vi "Resolve Type.vi"(8 "error in":errorcluster, 11 "Type Name":string) -> (0 "error out":errorcluster, 3 "Runtime Type":refnum<k24>)   [LabVIEW 2026, in "ToastNotification.lvlib" / "Reflection DotNet.lvlib"]
doc: "Resolve a runtime type by its assembly-qualified name using System.Type.GetType(name, true). Skipped on incoming error. The caller owns the returned System.Type reference. WinRT names can include ContentType=WindowsRuntime."
uses:
  Reflection DotNet.lvlib
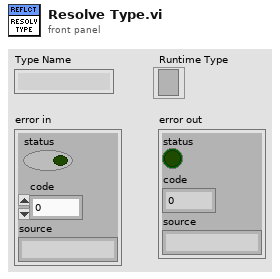
[diagram p1: front panel]
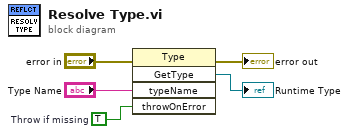
[diagram p0: block diagram]
diagram:
  w1 = TRUE  # Throw if missing
  n1 = invoke class="Type" method="GetType"(error in="error in", "typeName"="Type Name", "throwOnError"=w1) -> (error out=→"error out":errorcluster, "GetType"=→"Runtime Type":refnum<k24>)  [unwired: 2 in, 3 out]
